vi "TCP_Curve_Control(SubVI).vi"(0 "Tab mode":sgl, 1 "Speed Max":dbl, 2 "Step/s":dbl, 3 "Speed Mini":dbl, 4 "Theta Max":dbl, 5 "User Input Theta":dbl, 6 "Theta Mini":dbl, 7 "Jog Theta":sgl, 8 "Real Output Phi Ref":refnum<vi>, 9 "Phi Max":dbl, 10 "User Input Phi Ref":refnum<vi>, 11 "User Input Phi":dbl, 12 "Real Output Theta Ref":refnum<vi>, 13 "Phi Mini":dbl, 14 "User Input Theta Ref":refnum<vi>, 15 "Jog Phi":sgl, 16 "Moving R Ref":refnum<vi>, 17 "Tab Control Ref":refnum<vi>, 18 "Moving L Ref":refnum<vi>, 19 "Step/s Ref":refnum<vi>) -> (20 "Moving":bool, 21 "Real Output Theta":dbl, 22 "Real Output  Phi":dbl, 23 "TCP Left":bool, 24 "TCP Right":bool, 25 "TCP Up":bool, 26 "TCP Down":bool)   [LabVIEW 2018]
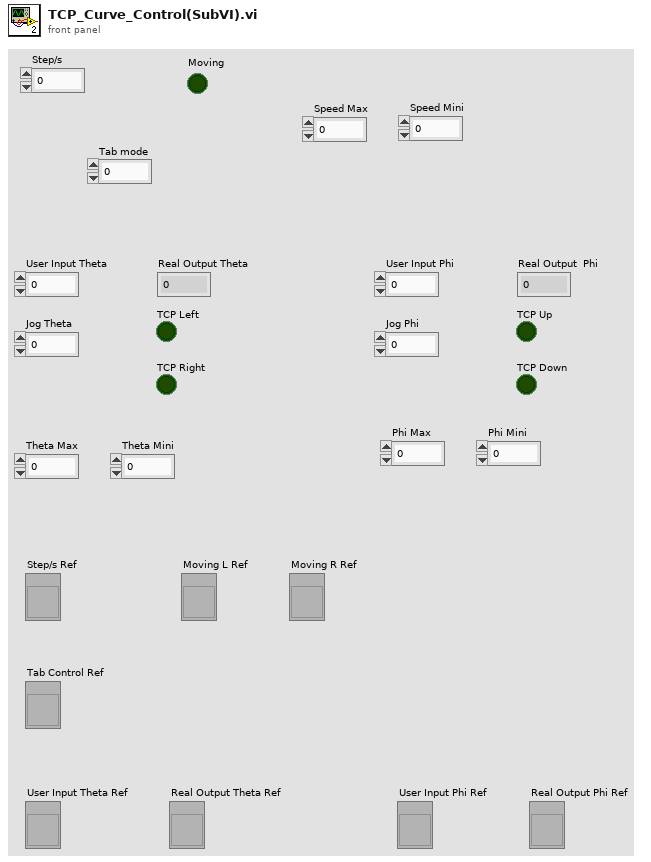
[diagram p1: front panel]
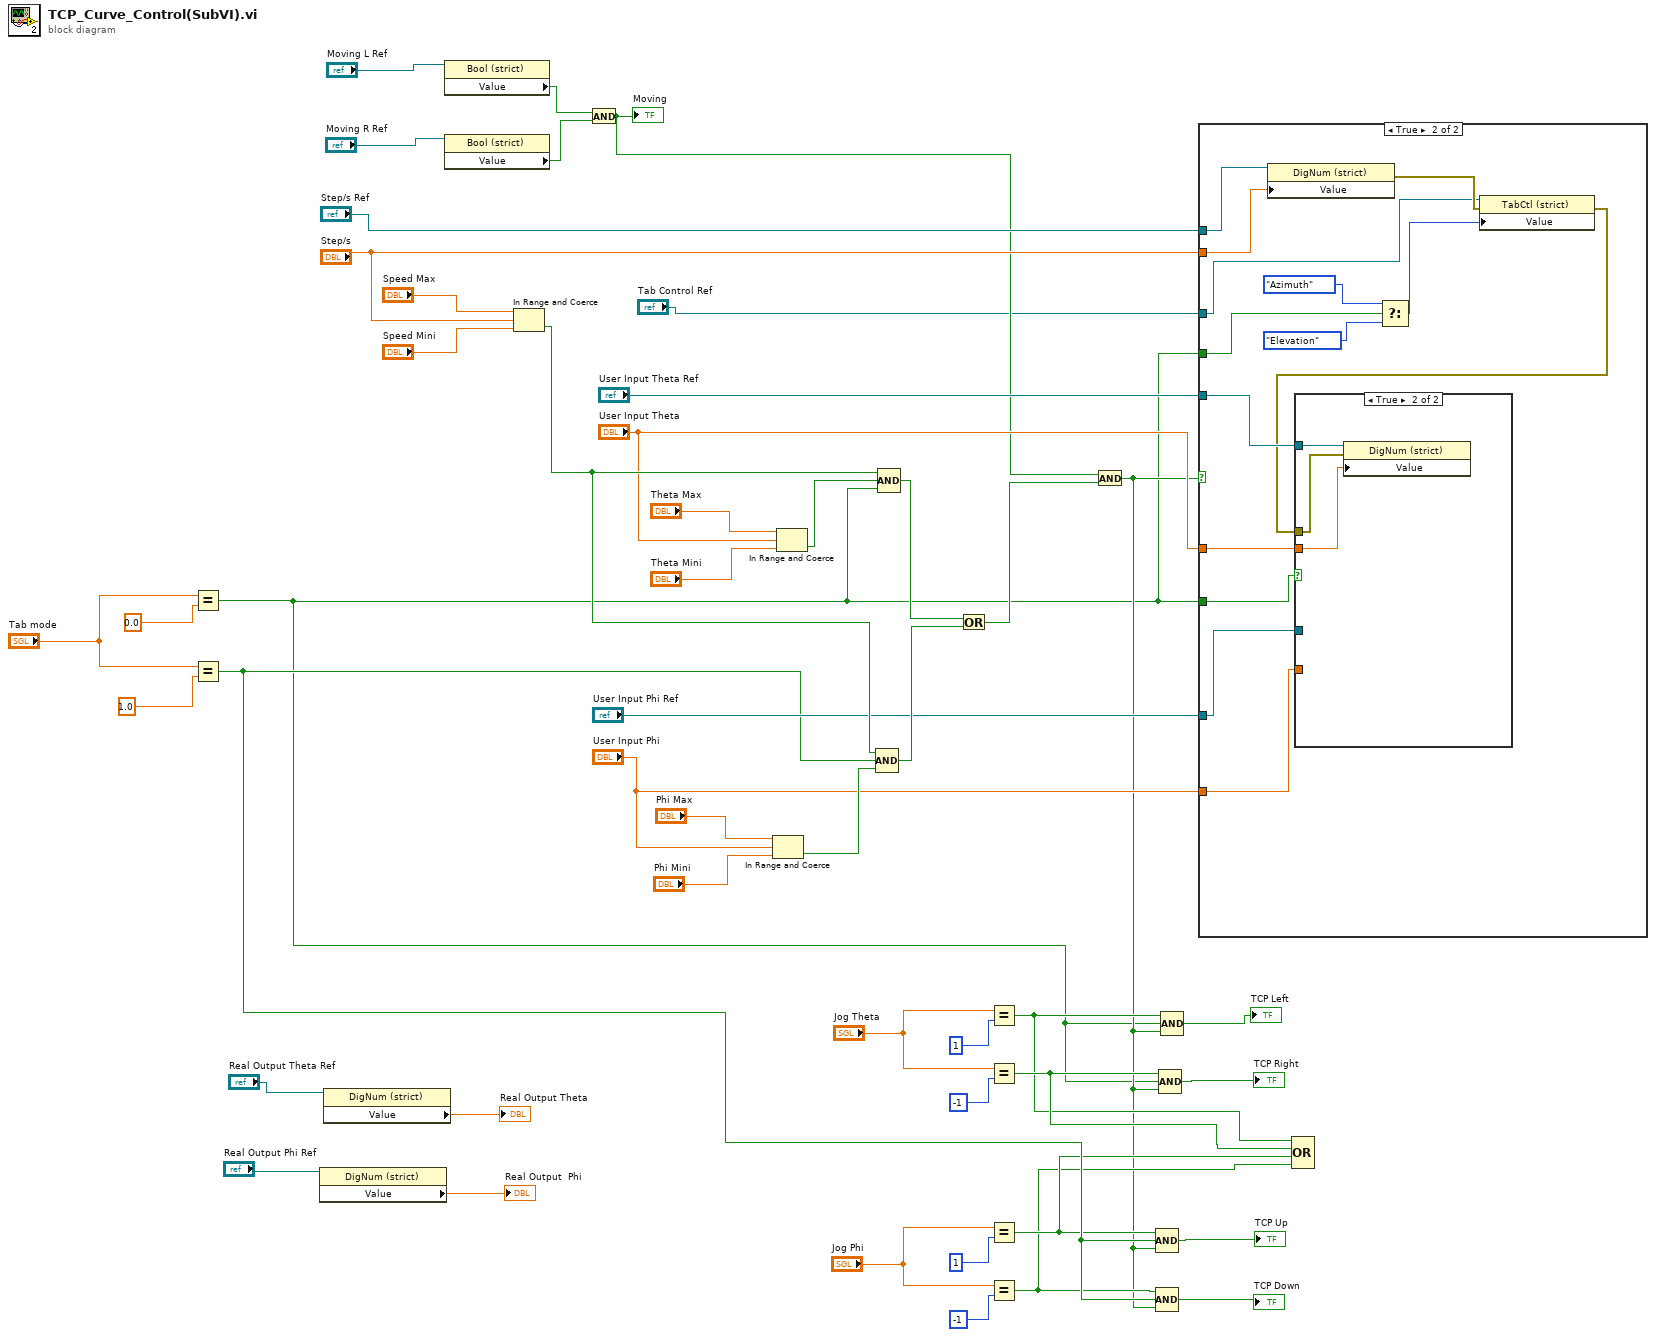
[diagram p0: block diagram]
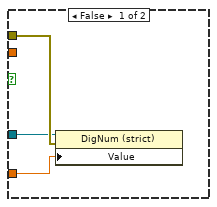
[diagram p3: hidden frame]
diagram:
  n1 = Equal?(x="Tab mode", y=0.0) -> (x = y?=w1:bool)
  n2 = Equal?(x="Tab mode", y=1.0) -> (x = y?=w16:bool)
  n3 = property class="DigNum (strict)"(reference="Real Output Phi Ref") -> ("Value"=→"Real Output  Phi":dbl)  [unwired: 1 in, 2 out]
  n4 = property class="DigNum (strict)"(reference="Real Output Theta Ref") -> ("Value"=→"Real Output Theta":dbl)  [unwired: 1 in, 2 out]
  n5 = property class="Bool (strict)"(reference="Moving L Ref") -> ("Value"=w5:bool)  [unwired: 1 in, 2 out]
  n6 = property class="Bool (strict)"(reference="Moving R Ref") -> ("Value"=w4:bool)  [unwired: 1 in, 2 out]
  n7 = In Range and Coerce(upper limit="Speed Max", x="Step/s", lower limit="Speed Mini") -> (In Range?=w23:bool)  [unwired: 1 out]
  n8 = And(x=w5, y=w4) -> (x .and. y?=w3:bool)
  "Moving" <- w3
  n9 = In Range and Coerce(upper limit="Phi Max", x="User Input Phi", lower limit="Phi Mini") -> (In Range?=w24:bool)  [unwired: 1 out]
  n10 = In Range and Coerce(upper limit="Theta Max", x="User Input Theta", lower limit="Theta Mini") -> (In Range?=w43:bool)  [unwired: 1 out]
  n11 = Compound Arithmetic op=AND(w23, w16, w24) -> (w21:bool)
  n12 = Compound Arithmetic op=AND(w23, w43, w1) -> (w22:bool)
  n13 = Or(x=w22, y=w21) -> (x .or. y?=w6:bool)
  n14 = Equal?(x="Jog Theta", y=1) -> (x = y?=w8:bool)
  n15 = Equal?(x="Jog Theta", y=-1) -> (x = y?=w9:bool)
  n16 = Equal?(x="Jog Phi", y=1) -> (x = y?=w11:bool)
  n17 = Equal?(x="Jog Phi", y=-1) -> (x = y?=w10:bool)
  n18 = And(x=w3, y=w6) -> (x .and. y?=w7:bool)
  n19 = Compound Arithmetic op=AND(w11, w16, w7) -> (→"TCP Up":bool)
  n20 = Compound Arithmetic op=AND(w10, w16, w7) -> (→"TCP Down":bool)
  n21 = Compound Arithmetic op=AND(w9, w1, w7) -> (→"TCP Right":bool)
  n22 = Compound Arithmetic op=AND(w8, w1, w7) -> (→"TCP Left":bool)
  n23 = case shown="True" w7 {
    tunnel: "Step/s Ref" -> [_ w62]
    tunnel: "Step/s" -> [_ w61]
    tunnel: "User Input Theta Ref" -> [_ w57]
    tunnel: "User Input Theta" -> [_ w55]
    tunnel: "User Input Phi Ref" -> [_ w56]
    tunnel: "User Input Phi" -> [_ w54]
    tunnel: "Tab Control Ref" -> [_ w51]
    tunnel: w1 -> [_ w50]
    tunnel: w1 -> [_ w49]
    frame False {
    }
    frame True {
      n24 = property class="DigNum (strict)"(reference=w62, "Value"=w61) -> (error out=w53:errorcluster)  [unwired: 1 in, 1 out]
      n25 = Select(t=enum32{"Azimuth", "Elevation"}."Azimuth" ("Value"), s=w49, f=enum32{"Azimuth", "Elevation"}."Elevation" ("Value")) -> (s? t:f=w60:enum32{"Azimuth", "Elevation"})
      n26 = property class="TabCtl (strict)"(reference=w51, error in=w53, "Value"=w60) -> (error out=w52:errorcluster)  [unwired: 1 out]
      n27 = case shown="True" w50 {
        tunnel: w52 -> [w65 w68]
        tunnel: w57 -> [_ w67]
        tunnel: w56 -> [w64 _]
        tunnel: w55 -> [_ w66]
        tunnel: w54 -> [w63 _]
        frame False {
          n28 = property class="DigNum (strict)"(reference=w64, error in=w65, "Value"=w63) -> ()  [unwired: 2 out]
        }
        frame True {
          n29 = property class="DigNum (strict)"(reference=w67, error in=w68, "Value"=w66) -> ()  [unwired: 2 out]
        }
      }
    }
  }
  n30 = Compound Arithmetic op=OR(w8, w9, w11, w10) -> ()  [unwired: 1 out]
